vi "Select Group.vi"(8 "error in (no error)":errorcluster, 10 "Group (Empty = none)":string, 11 "Historian Charting Manager in":refnum<class "Historian Charting Manager.lvclass">) -> (0 "error out":errorcluster, 3 "Historian Charting Manager out":refnum<class "Historian Charting Manager.lvclass">)   [LabVIEW 2020, in "VolatusGUI.lvlib" / "Historian Charting Manager.lvclass"]
uses:
  Historian Charting Manager.lvclass
  Historian Charting Manager.lvclass/Historian Charting Manager.ctl
  Select Plot Group Data.ctl
  Plot Group Config.ctl
  X-Axis Type.ctl
  Plot Config.ctl
  Scale.ctl
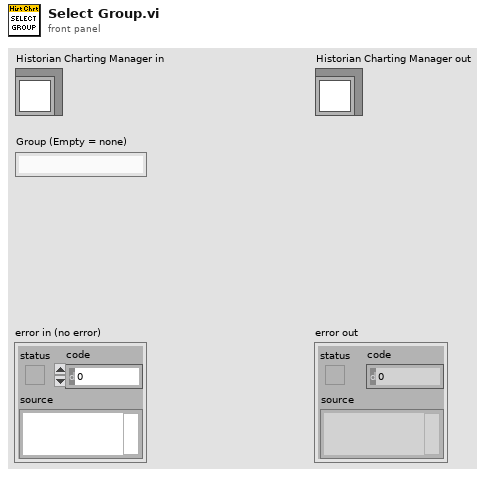
[diagram p1: front panel]
types:
  T1 = typedef "VolatusGUI.lvlib/Historian Charting Manager.lvclass/Plot Group Config.ctl" = cluster{"Name":string, "X-Axis Type":T2, "X-Axis Channel":string, "Plots":T3[], "Lock Now":bool, "Time":string, "Swap Axes":bool}
  T2 = typedef "VolatusGUI.lvlib/Historian Charting Manager.lvclass/X-Axis Type.ctl" = enum16{"Time", "Channel"}
  T3 = typedef "VolatusGUI.lvlib/Historian Charting Manager.lvclass/Plot Config.ctl" = cluster{"Channel":string, "Visible":bool, "Color":u32, "Scale":T4}
  T4 = typedef "VolatusGUI.lvlib/Historian Charting Manager.lvclass/Scale.ctl" = enum16{"Left", "Right"}
  T5 = typedef "VolatusGUI.lvlib/Historian Charting Manager.lvclass/Chart Info.ctl" = cluster{"PluginGUI":refnum<class "MessageQ.lvclass">, "Select Plot Group":refnum<user-event>}
  T6 = typedef "VolatusGUI.lvlib/Historian Charting Manager.lvclass/Select Plot Group Data.ctl" = cluster{"Chart Num":i32, "Plots Config":T1, "Plot Groups":string[]}
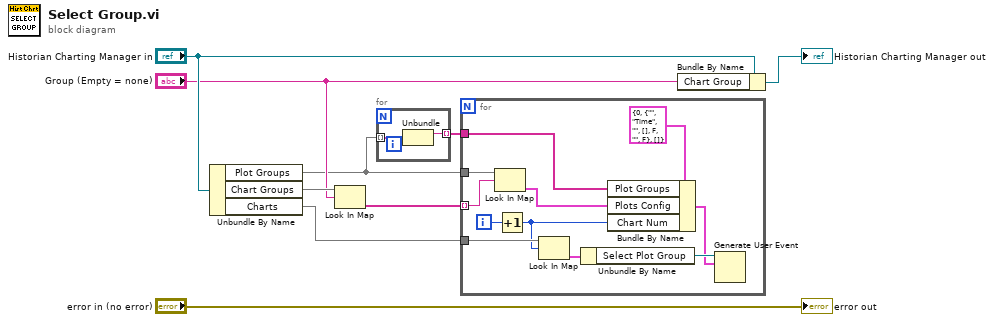
[diagram p0: block diagram]
diagram:
  n1 = Unbundle By Name("Historian Charting Manager in") -> ("Plot Groups"=w2:map{string, T1}, "Chart Groups"=w6:map{string, string[]}, "Charts"=w3:map{i32, T5})
  n2 = Look In Map(map=w6, key="Group (Empty = none)") -> (value=w4:string[])  [unwired: 1 in, 1 out]
  n3 = for {
    tunnel: w2 -> [w11] mode=indexing
    tunnel: [w10] -> w1 mode=indexing
    n4 = Unbundle(w11) -> ("Name"=w10:string)  [unwired: 1 out]
  }
  n5 = for {
    tunnel: w4 -> [w17] mode=indexing
    tunnel: w2 -> [w18]
    tunnel: w3 -> [w21]
    tunnel: w1 -> [w12]
    i -> [w22]
    n6 = Look In Map(map=w18, key=w17) -> (value=w14:T1)  [unwired: 1 in, 1 out]
    n7 = Increment(x=w22) -> (x+1=w13:i32)
    n8 = Look In Map(map=w21, key=w13) -> (value=w20:T5)  [unwired: 1 in, 1 out]
    n9 = Unbundle By Name(w20) -> ("Select Plot Group"=w19:refnum<user-event>)
    n10 = Bundle By Name(cluster=T6 {"Chart Num"=0, "Plots Config"={"Name"="", "X-Axis Type"=enum."Time", "X-Axis Channel"="", "Plots"=[], "Lock Now"=FALSE, "Time"="", "Swap Axes"=FALSE}, "Plot Groups"=[]} ("event data"), "Plot Groups"=w12, "Plots Config"=w14, "Chart Num"=w13) -> (w15:T6)
    n11 = Generate User Event(user event=w19, event data cluster=w15) -> ()  [unwired: 2 in, 2 out]
  }
  n12 = Bundle By Name(cluster="Historian Charting Manager in", "Chart Group"="Group (Empty = none)") -> (→"Historian Charting Manager out":refnum<class "Historian Charting Manager.lvclass">)
  "error out" <- "error in (no error)"
